vi "Config User Timestamps FIFO.vi"(8 "error in (no error)":errorcluster, 10 "Buffer Size (elements)":u32=1048576, 11 "FPGA Ref in":refnum<k20>) -> (0 "error out":errorcluster, 3 "FPGA Ref out":refnum<k20>)   [LabVIEW 2025, in "I2C Bus Monitor.lvclass"]
uses:
  I2C Bus Monitor.lvclass
  <vilib>/rvi/interface/common/niFpgaWaitOnOcc.vi
  <vilib>/Utility/error.llb/Error Cluster From Error Code.vi
  <vilib>/rvi/interface/nirviMethod/nirviMethod.xnode
  I2C Bus Monitor.lvclass/I2C Bus Monitor.ctl
  <vilib>/FPGAPlugInAG/Dynamic/niLvFpga_ConfigureFifo_Dynamic.vi
  <vilib>/rvi/errors/niLvFpgaMergeErrorWithErrorCode.vi
  <vilib>/FPGAPlugInAG/Dynamic/niLvFpga_StartFifo_Dynamic.vi
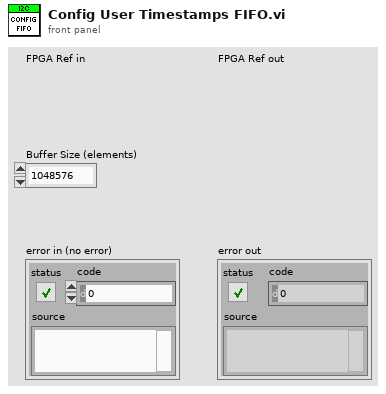
[diagram p1: front panel]
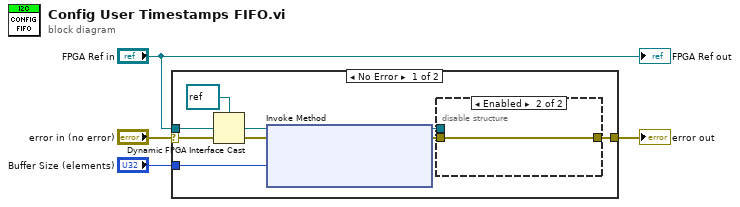
[diagram p0: block diagram]
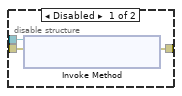
[diagram p2: hidden frame]
diagram:
  n1 = case shown="No Error" "error in (no error)" {
    selector: "error in (no error)" -> [w9 w17]
    tunnel: "Buffer Size (elements)" -> [w12 _]
    tunnel: [w11 w17] -> w3
    tunnel: "FPGA Ref in" -> [w5 _]
    frame No Error {
      n2 = Dynamic FPGA Interface Cast(Session In=refnum<k20> refnum ("FPGA VI Reference Out"), Type=w5) -> (Session Out=w7:refnum<k20>)
      n3 = xnode "Invoke Method"("FPGA VI Reference In"=w7, "error in"=w9, "Requested Depth"=w12) -> ("FPGA VI Reference Out"=w8:refnum<k20>, "error out"=w10:errorcluster)  [unwired: 1 out]
      n4 = disable-structure shown="Enabled" {
        disable-tunnel: [w15 w16] -> w11
        disable-tunnel: w10 -> [w14 w16]
        disable-tunnel: w8 -> [w13 _]
        frame Disabled {
          n5 = xnode "Invoke Method"("FPGA VI Reference In"=w13, "error in"=w14) -> ("error out"=w15:errorcluster)  [unwired: 1 out]
        }
        frame Enabled {
        }
      }
    }
    frame Error {
    }
  }
  "error out" <- w3
  "FPGA Ref out" <- "FPGA Ref in"
